vi "BC_list_selection.vi"(5 "BC_selection":u16(ring) items=["000.csv", "001.csv", "002.csv", "003.csv", "004.csv", "005.csv", "006.csv", "007.csv", "008.csv", "009.csv", "010_RNA_konno.csv", "011_Hitachi.csv", "012_Amino_AAbase (大城敬人 の競合コピー 2026-09-30).csv", "012_Amino_AAbase.csv"], 8 "error in":errorcluster) -> (0 "error out":errorcluster, 1 "path":string, 2 "Cluster":T1={"Right Read MIN"=6, "STD Type"=enum."Region", "Selection"=enum."10kHz", "Filter P"=0, "noise MAX"=3}, 3 "Base All Composition":T2(array[cluster]))   [LabVIEW 2018]
panel:
  out "concatenated string":string
  in  "Go Net":bool
  out "logical OR":bool
  out "Item":T3
  out "R STD Level":dbl
  out "R Base Level":dbl
  out "Base Color":u32
  out "ex":string
  out "Base Species IDX":i32
  out "path 2":path
  out "filenames":string[](array[string])
  out "path":path
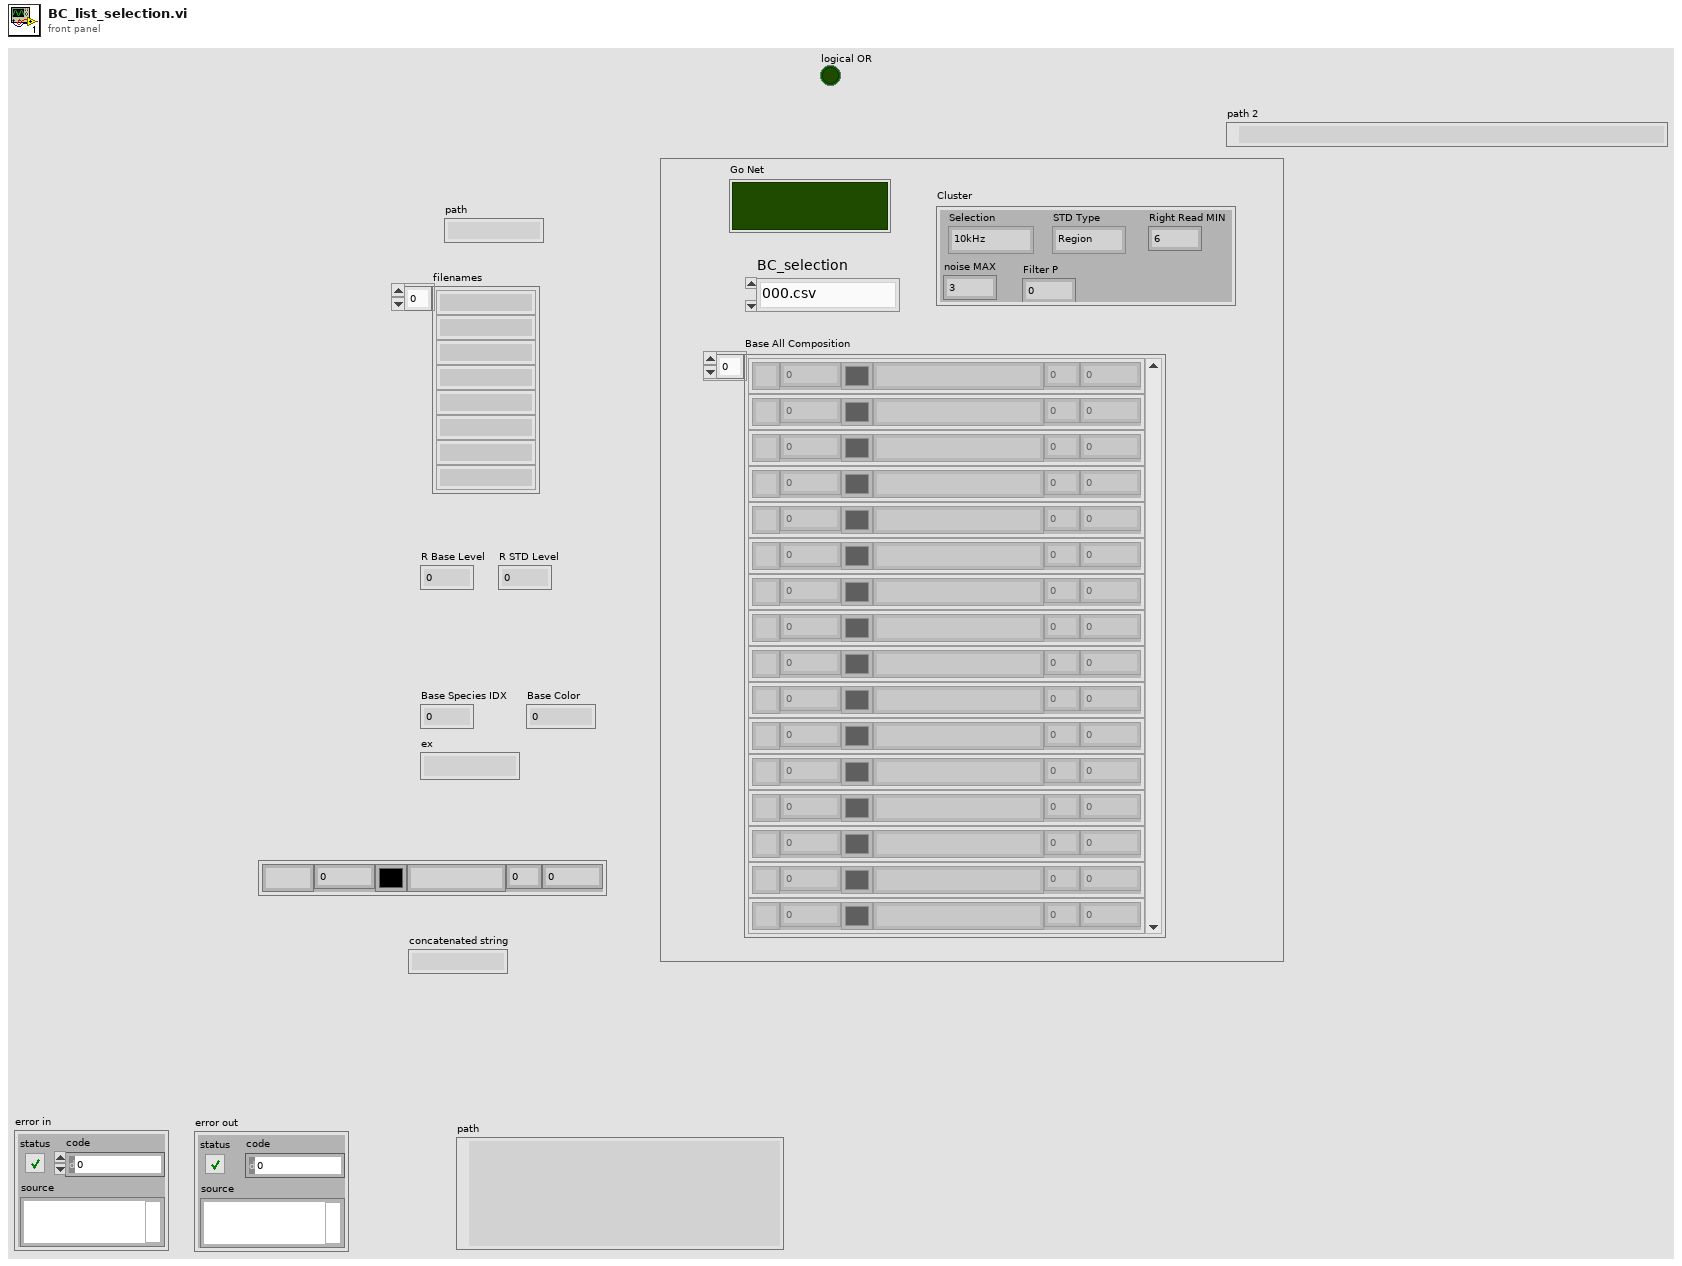
[diagram p1: front panel]
types:
  T1 = cluster{"Right Read MIN":i32, "STD Type":enum16{"Region", "Each", "Fixed"}, "Selection":enum16{"10kHz", "100kHz"}, "Filter P":i32, "noise MAX":i32}
  T2 = cluster{"Name":string, "Value":dbl, "Color":u32, "Name 2":string, "Value 2":dbl, "Value 3":dbl}[]
  T3 = cluster{"Name":string, "Value":dbl, "Color":u32, "Name 2":string, "Value 2":dbl, "Value 3":dbl}
  T4 = cluster{"String":string, dbl, i32, "String":string, i32, dbl}
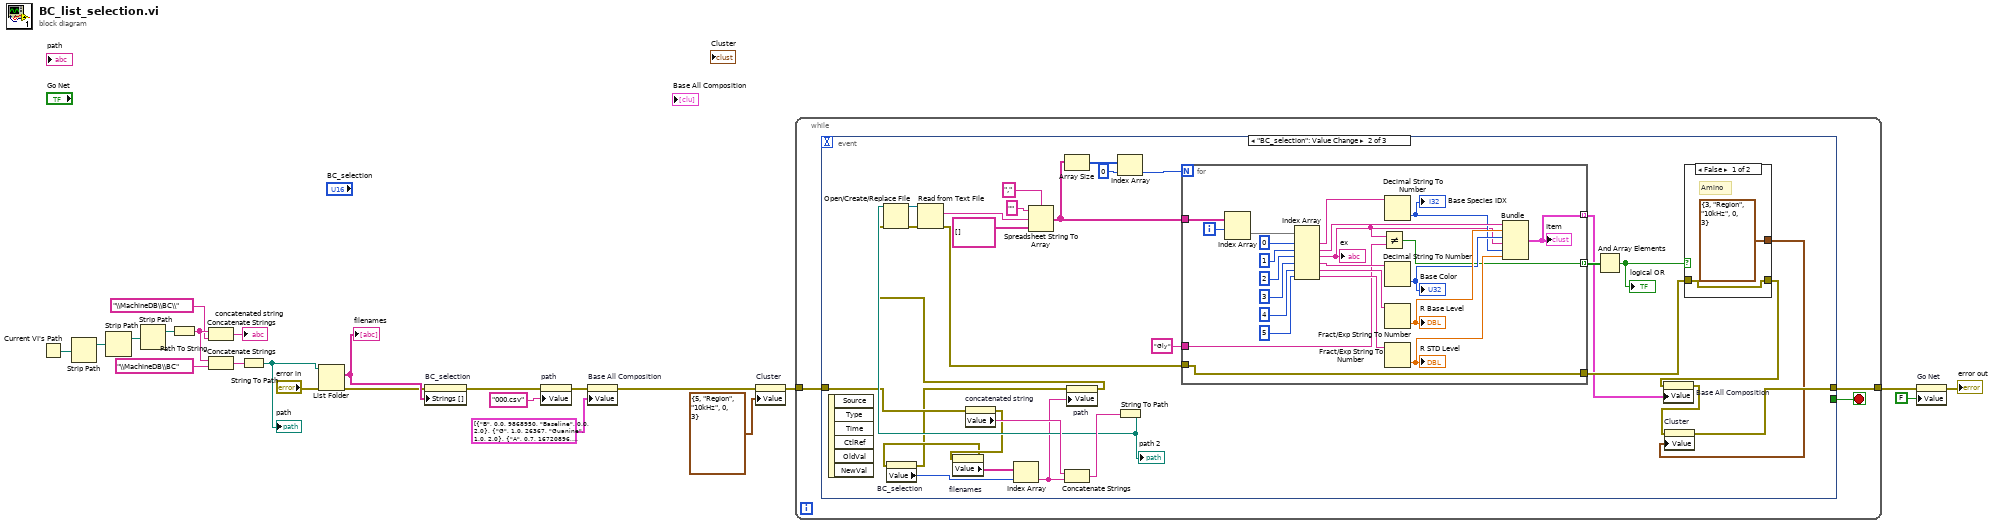
[diagram p0: block diagram]
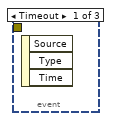
[diagram p2: hidden frame]
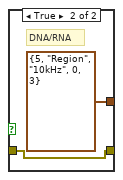
[diagram p3: hidden frame]
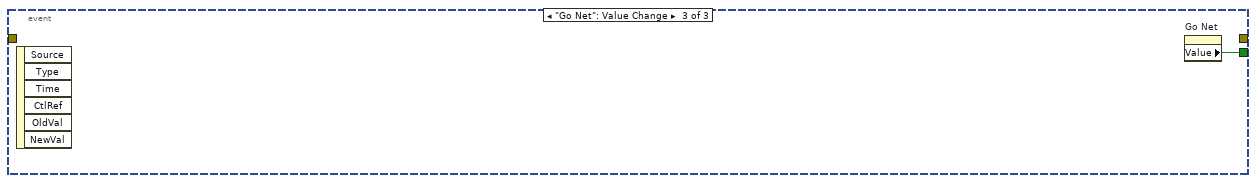
[diagram p4: hidden frame]
diagram:
  n1 = Current VI's Path() -> (path=w23:path)
  n2 = Strip Path(path=w23) -> (stripped path=w22:path)  [unwired: 1 out]
  n3 = Strip Path(path=w22) -> (stripped path=w21:path)  [unwired: 1 out]
  n4 = Strip Path(path=w21) -> (stripped path=w20:path)  [unwired: 1 out]
  n5 = Path To String(path=w20) -> (string=w4:string)
  n6 = Concatenate Strings(w4, "\\MachineDB\\BC\\" ("string")) -> (→"concatenated string":string)
  n7 = Concatenate Strings(w4, "\\MachineDB\\BC" ("string")) -> (w15:string)
  n8 = String To Path(string=w15) -> (path=w18:path)
  "path" <- w18
  n9 = List Folder(path=w18, error in="error in") -> (filenames=w17:string[], error out=w16:errorcluster)  [unwired: 2 in, 2 out]
  "filenames" <- w17
  n10 = property on="BC_selection" class="Ring (strict)"(error in=w16, "Strings []"=w17) -> (error out=w8:errorcluster)  [unwired: 1 in, 1 out]
  n11 = property on="path" class="Str"(error in=w8, "Value"="000.csv" ("path")) -> (error out=w6:errorcluster)  [unwired: 1 in, 1 out]
  n12 = property on="Base All Composition" class="Arr (strict)"(error in=w6, "Value"=T2 [{"Name"="B", "Value"=0.0, "Color"=9868950, "Name 2"="Baseline", "Value 2"=0.0, "Value 3"=2.0}, {"Name"="G", "Value"=1.0, "Color"=26367, "Name 2"="Guanine", "Value 2"=1.0, "Value 3"=2.0}, {"Name"="A", "Value"=0.7, "Color"=16720896, "Name 2"="Adenine", "Value 2"=2.0, "Value 3"=2.0}, {"Name"="C", "Value"=0.6, "Color"=12397311, "Name 2"="Cytosine", "Value 2"=3.0, "Value 3"=2.0}, {"Name"="T", "Value"=0.23, "Color"=6618880, "Name 2"="Thymine", "Value 2"=4.0, "Value 3"=2.0}, {"Name"="U", "Value"=0.38, "Color"=5898210, "Name 2"="Uracil", "Value 2"=5.0, "Value 3"=2.0}, {"Name"="M", "Value"=1.2, "Color"=16472575, "Name 2"="5-Methlycytosine", "Value 2"=6.0, "Value 3"=2.0}, {"Name"="N", "Value"=0.9, "Color"=15698688, "Name 2"="N6-Methlyadenine", "Value 2"=7.0, "Value 3"=2.0}, {"Name"="H", "Value"=0.82, "Color"=6291695, "Name 2"="5-Hydroxymethlycytosine", "Value 2"=8.0, "Value 3"=2.0}, {"Name"="F", "Value"=0.2, "Color"=16772608, "Name 2"="Trifluridine (TFT)", "Value 2"=9.0, "Value 3"=2.0}, {"Name"="W", "Value"=0.18, "Color"=16761088, "Name 2"="Fluorouracil (5FU)", "Value 2"=10.0, "Value 3"=2.0}, {"Name"="X", "Value"=1.4, "Color"=16771535, "Name 2"="Unknown 1", "Value 2"=11.0, "Value 3"=2.0}, {"Name"="Y", "Value"=1.2, "Color"=8016737, "Name 2"="Unknown 2", "Value 2"=12.0, "Value 3"=2.0}, {"Name"="Z", "Value"=0.957, "Color"=11776947, "Name 2"="Unknown 3", "Value 2"=13.0, "Value 3"=2.0}] ("Base All Composition 2")) -> (error out=w5:errorcluster)  [unwired: 1 in, 1 out]
  n13 = property on="Cluster" class="Clust (strict)"(error in=w5, "Value"=T1 {"Right Read MIN"=5, "STD Type"=enum."Region", "Selection"=enum."10kHz", "Filter P"=0, "noise MAX"=3} ("Cluster 2")) -> (error out=w1:errorcluster)  [unwired: 1 in, 1 out]
  n14 = while {
    tunnel: [w25] -> w13
    tunnel: w1 -> [w24]
    stop <- w26 stop-if-true
    n15 = event shown="[1] \"BC_selection\": Value Change" {
      selector: _ -> [_ _ _]
      dyn-events: _ -> [_ _ _]
      timeout: _ -> [_ _ _]
      tunnel: [_ _ w85] -> w26
      tunnel: [_ w33 _] -> w25
      tunnel: w24 -> [_ w39 _]
      event Timeout {
        n16 = event-data() -> ()  [unwired: 1 in, 3 out]
      }
      event "BC_selection": Value Change {
        n17 = event-data() -> ()  [unwired: 1 in, 6 out]
        n18 = property on="concatenated string" class="Str"(error in=w39) -> (error out=w38:errorcluster, "Value"=w55:string)  [unwired: 1 in, 1 out]
        n19 = property on="filenames" class="Arr (strict)"(error in=w38) -> (error out=w37:errorcluster, "Value"=w57:string[])  [unwired: 1 in, 1 out]
        n20 = property on="BC_selection" class="Ring (strict)"(error in=w37) -> (error out=w28:errorcluster, "Value"=w56:u16)  [unwired: 1 in, 1 out]
        n21 = Index Array(array=w57, index=w56) -> (element=w29:string)
        n22 = Concatenate Strings(w55, w29) -> (w41:string)
        n23 = property on="path" class="Str"(error in=w28, "Value"=w29) -> (error out=w27:errorcluster)  [unwired: 1 in, 1 out]
        n24 = String To Path(string=w41) -> (path=w40:path)
        "path 2" <- w40
        n25 = Open/Create/Replace File(file path (use dialog)=w40, error in=w27) -> (refnum out=w48:refnum<file>, error out=w47:errorcluster)  [unwired: 4 in, 1 out]
        n26 = Read from Text File(file (use dialog)=w48, error in=w47) -> (text=w49:string, error out=w36:errorcluster)  [unwired: 2 in, 2 out]
        n27 = Spreadsheet String To Array(delimiter (Tab)=",", format string="", spreadsheet string=w49, array type (2D Dbl)=string[][] []) -> (array=w50:string[][])
        n28 = Array Size(array=w50) -> (size(s)=w51:i32[])
        n29 = Index Array(array=w51, index=0) -> (element=w52:i32)
        n30 = for {
          N: w52 -> [_]
          tunnel: w50 -> [w68]
          tunnel: [w66] -> w32 mode=indexing
          tunnel: "Gly" -> [w65]
          tunnel: [w63] -> w53 mode=indexing
          tunnel: w36 -> [w62]
          tunnel: [w62] -> w35
          i -> [w67]
          n31 = Index Array(array=w68, index (row)=w67) -> (element=w84:string[])  [unwired: 1 in]
          n32 = Index Array(array=w84, index #1=0 ("index"), index #2=1 ("index"), index #3=2 ("index"), index #4=3 ("index"), index #5=4 ("index"), index #6=5 ("index")) -> (element #1=w82:string, element #2=w80:string, element #3=w64:string, element #4=w74:string, element #5=w76:string, element #6=w71:string)
          "ex" <- w64
          n33 = Not Equal?(x=w64, y=w65) -> (x != y?=w63:bool)
          n34 = Decimal String To Number(string=w82) -> (number=w70:i32)  [unwired: 2 in, 1 out]
          "Base Species IDX" <- w70
          n35 = Decimal String To Number(string=w74) -> (number=w73:i32)  [unwired: 2 in, 1 out]
          "Base Color" <- w73
          n36 = Fract/Exp String To Number(string=w76) -> (number=w75:dbl)  [unwired: 3 in, 1 out]
          "R Base Level" <- w75
          n37 = Fract/Exp String To Number(string=w71) -> (number=w69:dbl)  [unwired: 3 in, 1 out]
          "R STD Level" <- w69
          n38 = Bundle("String"=w80, w75, w73, "String"=w64, w70, w69) -> (w66:T4)  [unwired: 1 in]
          "Item" <- w66
        }
        n39 = And Array Elements(Boolean array=w53) -> (logical AND=w54:bool)
        "logical OR" <- w54
        n40 = case shown="False" w54 {
          tunnel: [T1 {"Right Read MIN"=3, "STD Type"=enum."Region", "Selection"=enum."10kHz", "Filter P"=0, "noise MAX"=3} ("Cluster 2") T1 {"Right Read MIN"=5, "STD Type"=enum."Region", "Selection"=enum."10kHz", "Filter P"=0, "noise MAX"=3} ("Cluster 2")] -> w30
          tunnel: w35 -> [w58 w60]
          tunnel: [w58 w60] -> w31
          frame False {
            # "Amino"
          }
          frame True {
            # "DNA/RNA"
          }
        }
        n41 = property on="Base All Composition" class="Arr (strict)"(error in=w31, "Value"=w32) -> (error out=w34:errorcluster)  [unwired: 1 in, 1 out]
        n42 = property on="Cluster" class="Clust (strict)"(error in=w34, "Value"=w30) -> (error out=w33:errorcluster)  [unwired: 1 in, 1 out]
      }
      event "Go Net": Value Change {
        n43 = event-data() -> ()  [unwired: 1 in, 6 out]
        n44 = property on="Go Net" class="Bool (strict)"() -> ("Value"=w85:bool)  [unwired: 2 in, 2 out]
      }
    }
  }
  n45 = property on="Go Net" class="Bool (strict)"(error in=w13, "Value"=FALSE ("Go Net")) -> (error out=→"error out":errorcluster)  [unwired: 1 in, 1 out]
